vi "Two Color Cal Get Image.vi"(0 "Notifier Name":string, 11 "Frames to Wait":u32) -> ()   [LabVIEW 2016]
uses:
  Device Library/Cameras/Camera Controls/Generic Camera Actions.ctl
  Device Library/Cameras/Camera Controls/Camera IMAQ Key Info.ctl
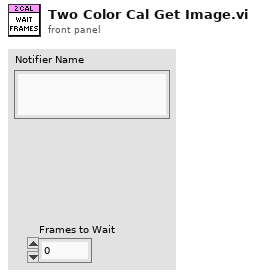
[diagram p1: front panel]
types:
  T1 = typedef "Generic Camera Actions.ctl" = enum16{"Status", "Live Preview", "Capture", "Abort", "Set Exposure Time (s)", "Get Exposure Time (s)", "Record Settings", "Set ROI", "Get ROI", "Defect Correction On/Off", "Cooler On/Off", "Fan On/Off", "Quti"}
  T2 = typedef "IMAQ Image.ctl" = refnum<image>
  T3 = typedef "Camera IMAQ Key Info.ctl" = cluster{"Frame":u32, "Sensor Height":i32, "Sensor Width":i32, "ROI Height":i32, "ROI Width":i32, "ROI Enable?":bool, "Bit per Pixel":u8}
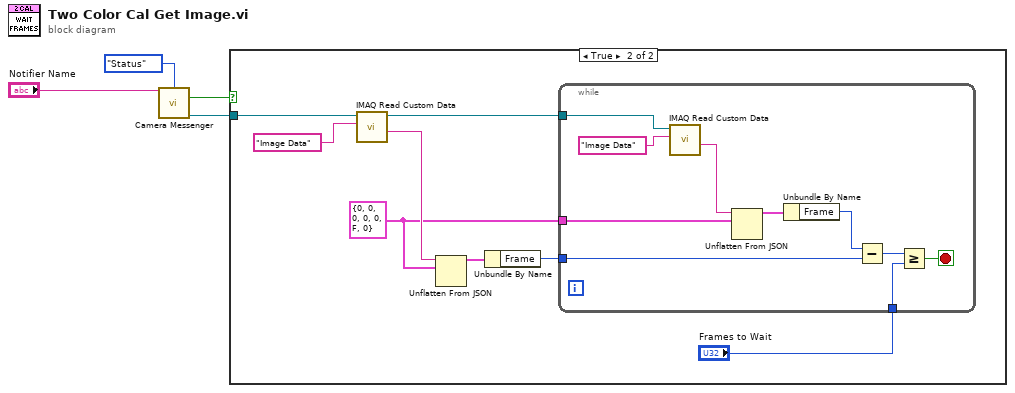
[diagram p0: block diagram]
diagram:
  n1 = call "Camera Messenger.vi"("Notifier Name"="Notifier Name", "General Camera Actions"=Generic_Camera_Actions."Status") -> ("Running?"=w1:bool, "Image Ref"=w3:T2)  [unwired: 8 in, 4 out]
  n2 = case shown="True" w1 {
    tunnel: w3 -> [_ w10]
    frame False {
    }
    frame True {
      w8 = T3 {"Frame"=0, "Sensor Height"=0, "Sensor Width"=0, "ROI Height"=0, "ROI Width"=0, "ROI Enable?"=FALSE, "Bit per Pixel"=0} ("Camera IMAQ Key Info")
      n3 = call "IMAQ Read Custom Data"("Key"="Image Data", "Image"=w10) -> ("Custom Data Out"=w12:string, "Image (duplicate)"=w7:T2)  [unwired: 7 in, 1 out]
      n4 = Unflatten From JSON(JSON string=w12, type and defaults=w8) -> (value=w9:T3)  [unwired: 5 in, 1 out]
      n5 = Unbundle By Name(w9) -> ("Frame"=w6:u32)
      n6 = while {
        tunnel: w7 -> [w18]
        tunnel: w8 -> [w19]
        tunnel: w6 -> [w16]
        tunnel: "Frames to Wait" -> [w14]
        stop <- w13 stop-if-true
        n7 = call "IMAQ Read Custom Data"("Key"="Image Data", "Image"=w18) -> ("Custom Data Out"=w21:string)  [unwired: 7 in, 2 out]
        n8 = Unflatten From JSON(JSON string=w21, type and defaults=w19) -> (value=w22:T3)  [unwired: 5 in, 1 out]
        n9 = Unbundle By Name(w22) -> ("Frame"=w17:u32)
        n10 = Subtract(x=w17, y=w16) -> (x-y=w15:u32)
        n11 = Greater Or Equal?(x=w15, y=w14) -> (x >= y?=w13:bool)
      }
    }
  }
